vi "MathUtil_ApplyDeadband.vi"(9 "Max Magnitude":dbl=1.0, 10 "Deadband":dbl=0.05, 11 "Value":dbl) -> (3 "Result":dbl)   [LabVIEW 2019, in "Trajectory_Library.lvlib"]
doc: "Returns 0.0 if the given value is within the specified range around zero. The remaining range between the deadband and the maximum magnitude is scaled from 0.0 to the maximum magnitude. \nInputs:\n - value -- Value to clip.\n - deadband -- Range around zero.\n - max magnitude -- The maximum magnitude of the input. Can be infinite. (Default: 1.0)\n\nOutputs:\n - Result -- The value after the deadband is applied."
uses:
  Trajectory_Library.lvlib
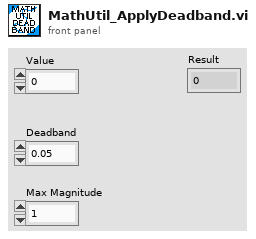
[diagram p1: front panel]
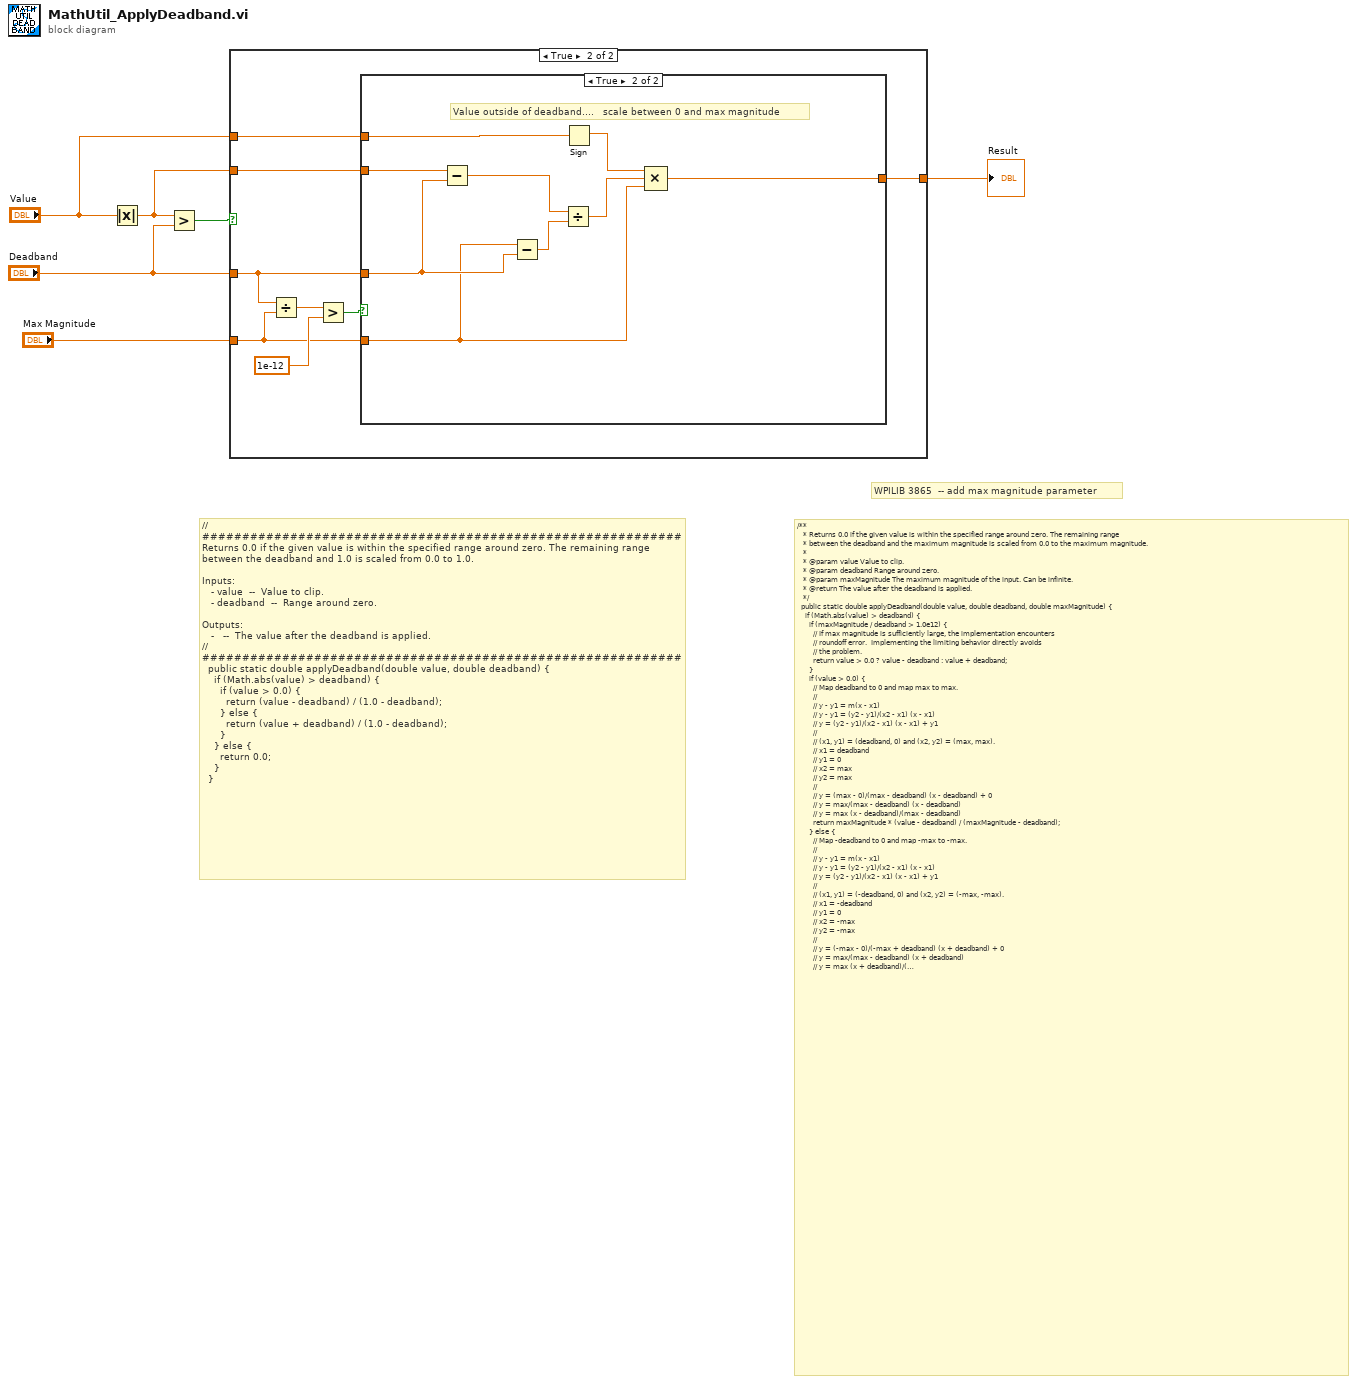
[diagram p0: block diagram]
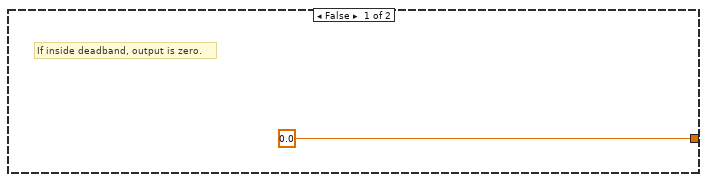
[diagram p2: hidden frame]
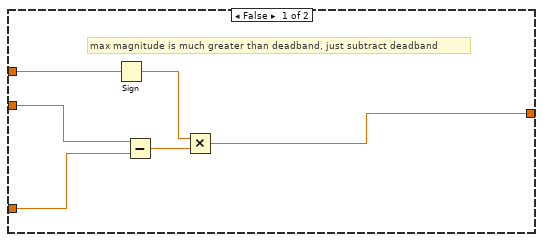
[diagram p3: hidden frame]
diagram:
  # "WPILIB 3865  -- add max magnitude parameter"
  # "/**\n   * Returns 0.0 if the given value is within the specified range around zero. The remaining range\n   * between the deadband and the maximum magnitude is scaled from 0.0 to the maximum magnitude.\n   *\n   * @param value Value to clip.\n   * @param deadband Range around zero.\n   * @param maxMagnitude The maximum magnitude of the input. Can be infinite.\n   * @return The value after the deadband is applied.\n   */\n  public static double applyDeadband(double value, double deadband, double maxMagnitude) {\n    if (Math.abs(value) > deadband) {\n      if (maxMagnitude / deadband > 1.0e12) {\n        // If max magnitude is sufficiently large, the implementation encounters\n        // roundoff error.  Implementing the limiting behavior directly avoids\n        // the problem.\n        return value > 0.0 ? value - deadband : value + deadband;\n      }\n      if (value > 0.0) {\n        // Map deadband to 0 and map max to max.\n        //\n        // y - y1 = m(x - x1)\n        // y - y1 = (y2 - y1)/(x2 - x1) (x - x1)\n        // y = (y2 - y1)/(x2 - x1) (x - x1) + y1\n        //\n        // (x1, y1) = (deadband, 0) and (x2, y2) = (max, max).\n        // x1 = deadband\n        // y1 = 0\n        // x2 = max\n        // y2 = max\n        //\n        // y = (max - 0)/(max - deadband) (x - deadband) + 0\n        // y = max/(max - deadband) (x - deadband)\n        // y = max (x - deadband)/(max - deadband)\n        return maxMagnitude * (value - deadband) / (maxMagnitude - deadband);\n      } else {\n        // Map -deadband to 0 and map -max to -max.\n        //\n        // y - y1 = m(x - x1)\n        // y - y1 = (y2 - y1)/(x2 - x1) (x - x1)\n        // y = (y2 - y1)/(x2 - x1) (x - x1) + y1\n        //\n        // (x1, y1) = (-deadband, 0) and (x2, y2) = (-max, -max).\n        // x1 = -deadband\n        // y1 = 0\n        // x2 = -max\n        // y2 = -max\n        //\n        // y = (-max - 0)/(-max + deadband) (x + deadband) + 0\n        // y = max/(max - deadband) (x + deadband)\n        // y = max (x + deadband)/(max - deadband)\n        return maxMagnitude * (value + deadband) / (maxMagnitude - deadband);\n      }\n    } else {\n      return 0.0;\n    }\n  }"
  # "//############################################################\nReturns 0.0 if the given value is within the specified range around zero. The remaining range\nbetween the deadband and 1.0 is scaled from 0.0 to 1.0.\n  \nInputs:\n   - value  --  Value to clip.\n   - deadband  --  Range around zero.\n\nOutputs:\n   -   --  The value after the deadband is applied.\n//############################################################\n  public static double applyDeadband(double value, double deadband) {\n    if (Math.abs(value) > deadband) {\n      if (value > 0.0) {\n        return (value - deadband) / (1.0 - deadband);\n      } else {\n        return (value + deadband) / (1.0 - deadband);\n      }\n    } else {\n      return 0.0;\n    }\n  }"
  n1 = Absolute Value(x="Value") -> (abs(x)=w4:dbl)
  n2 = Greater?(x=w4, y="Deadband") -> (0:w6:bool)
  n3 = case shown="True" w6 {
    tunnel: w4 -> [_ w15]
    tunnel: "Deadband" -> [_ w12]
    tunnel: "Value" -> [_ w14]
    tunnel: [0.0 w13] -> w2
    tunnel: "Max Magnitude" -> [_ w8]
    frame False {
      # "If inside deadband, output is zero."
    }
    frame True {
      n4 = Divide(x=w12, y=w8) -> (x/y=w11:dbl)
      n5 = Greater?(x=w11, y=1e-12) -> (0:w9:bool)
      n6 = case shown="True" w9 {
        tunnel: w15 -> [w21 w30]
        tunnel: w14 -> [w19 w27]
        tunnel: [w16 w24] -> w13
        tunnel: w12 -> [w20 w23]
        tunnel: w8 -> [_ w22]
        frame False {
          # "max magnitude is much greater than deadband, just subtract deadband"
          n7 = Sign(1:w19) -> (0:w18:dbl)
          n8 = Subtract(x=w21, y=w20) -> (x-y=w17:dbl)
          n9 = Multiply(x=w18, y=w17) -> (x*y=w16:dbl)
        }
        frame True {
          # "Value outside of deadband....   scale between 0 and max magnitude"
          n10 = Subtract(x=w30, y=w23) -> (x-y=w28:dbl)
          n11 = Subtract(x=w22, y=w23) -> (x-y=w29:dbl)
          n12 = Divide(x=w28, y=w29) -> (x/y=w26:dbl)
          n13 = Sign(1:w27) -> (0:w25:dbl)
          n14 = Compound Arithmetic op=MULTIPLY(w25, w26, w22) -> (w24:dbl)
        }
      }
    }
  }
  "Result" <- w2
